vi "Sequence Anal Tri_Di.vi"(8 "Level Composition":string[](array[string]), 11 "String":string="TCTAGACTATCTCACTCTCAGATGAGATCGATAGATCAGT") -> (0 "BaseNumber":cluster{i32[], i32[], i32[]}, 1 "B%Number":cluster{dbl[], dbl[], dbl[]}, 3 "Base Tag":T1)   [LabVIEW 2018]
panel:
  out "MonoBase_Array_Tag":string[](array[string])=["AC", "AT", "AG", "CA", "CG", "CT", "GA", "GC", "GT", "TA", "TC", "TG"]
  out "MonoBase_Array":i32[](array[numeric])
  out "Mono_Array":string[](array[string])
  out "TriBase_Array":i32[](array[numeric])
  out "TriBase_Array_Tag":string[](array[string])=["AC", "AT", "AG", "CA", "CG", "CT", "GA", "GC", "GT", "TA", "TC", "TG"]
  out "DiBase_Array_Tag":string[](array[string])=["AC", "AT", "AG", "CA", "CG", "CT", "GA", "GC", "GT", "TA", "TC", "TG"]
  out "DiBase_Array":i32[](array[numeric])
  out "TriBase_Array":string[](array[string])
  out "DiBase_Array":string[](array[string])
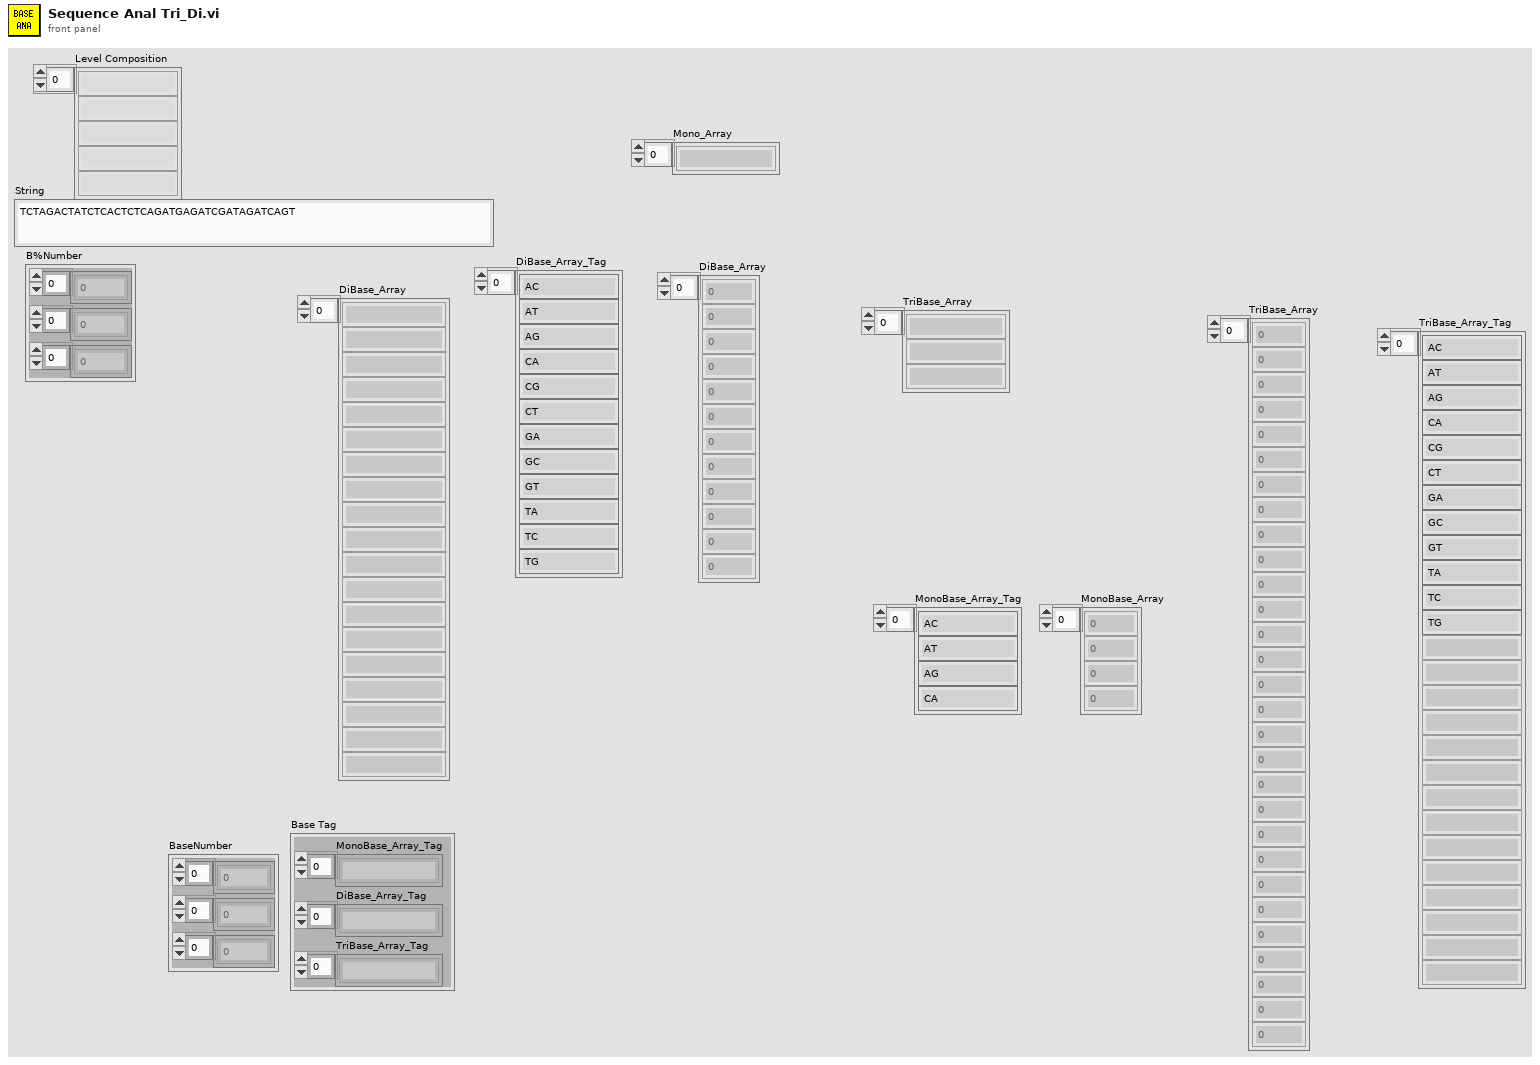
[diagram p1: front panel]
types:
  T1 = cluster{"MonoBase_Array_Tag":string[], "DiBase_Array_Tag":string[], "TriBase_Array_Tag":string[]}
  T2 = cluster{"Level Composition":string[], string[], string[]}
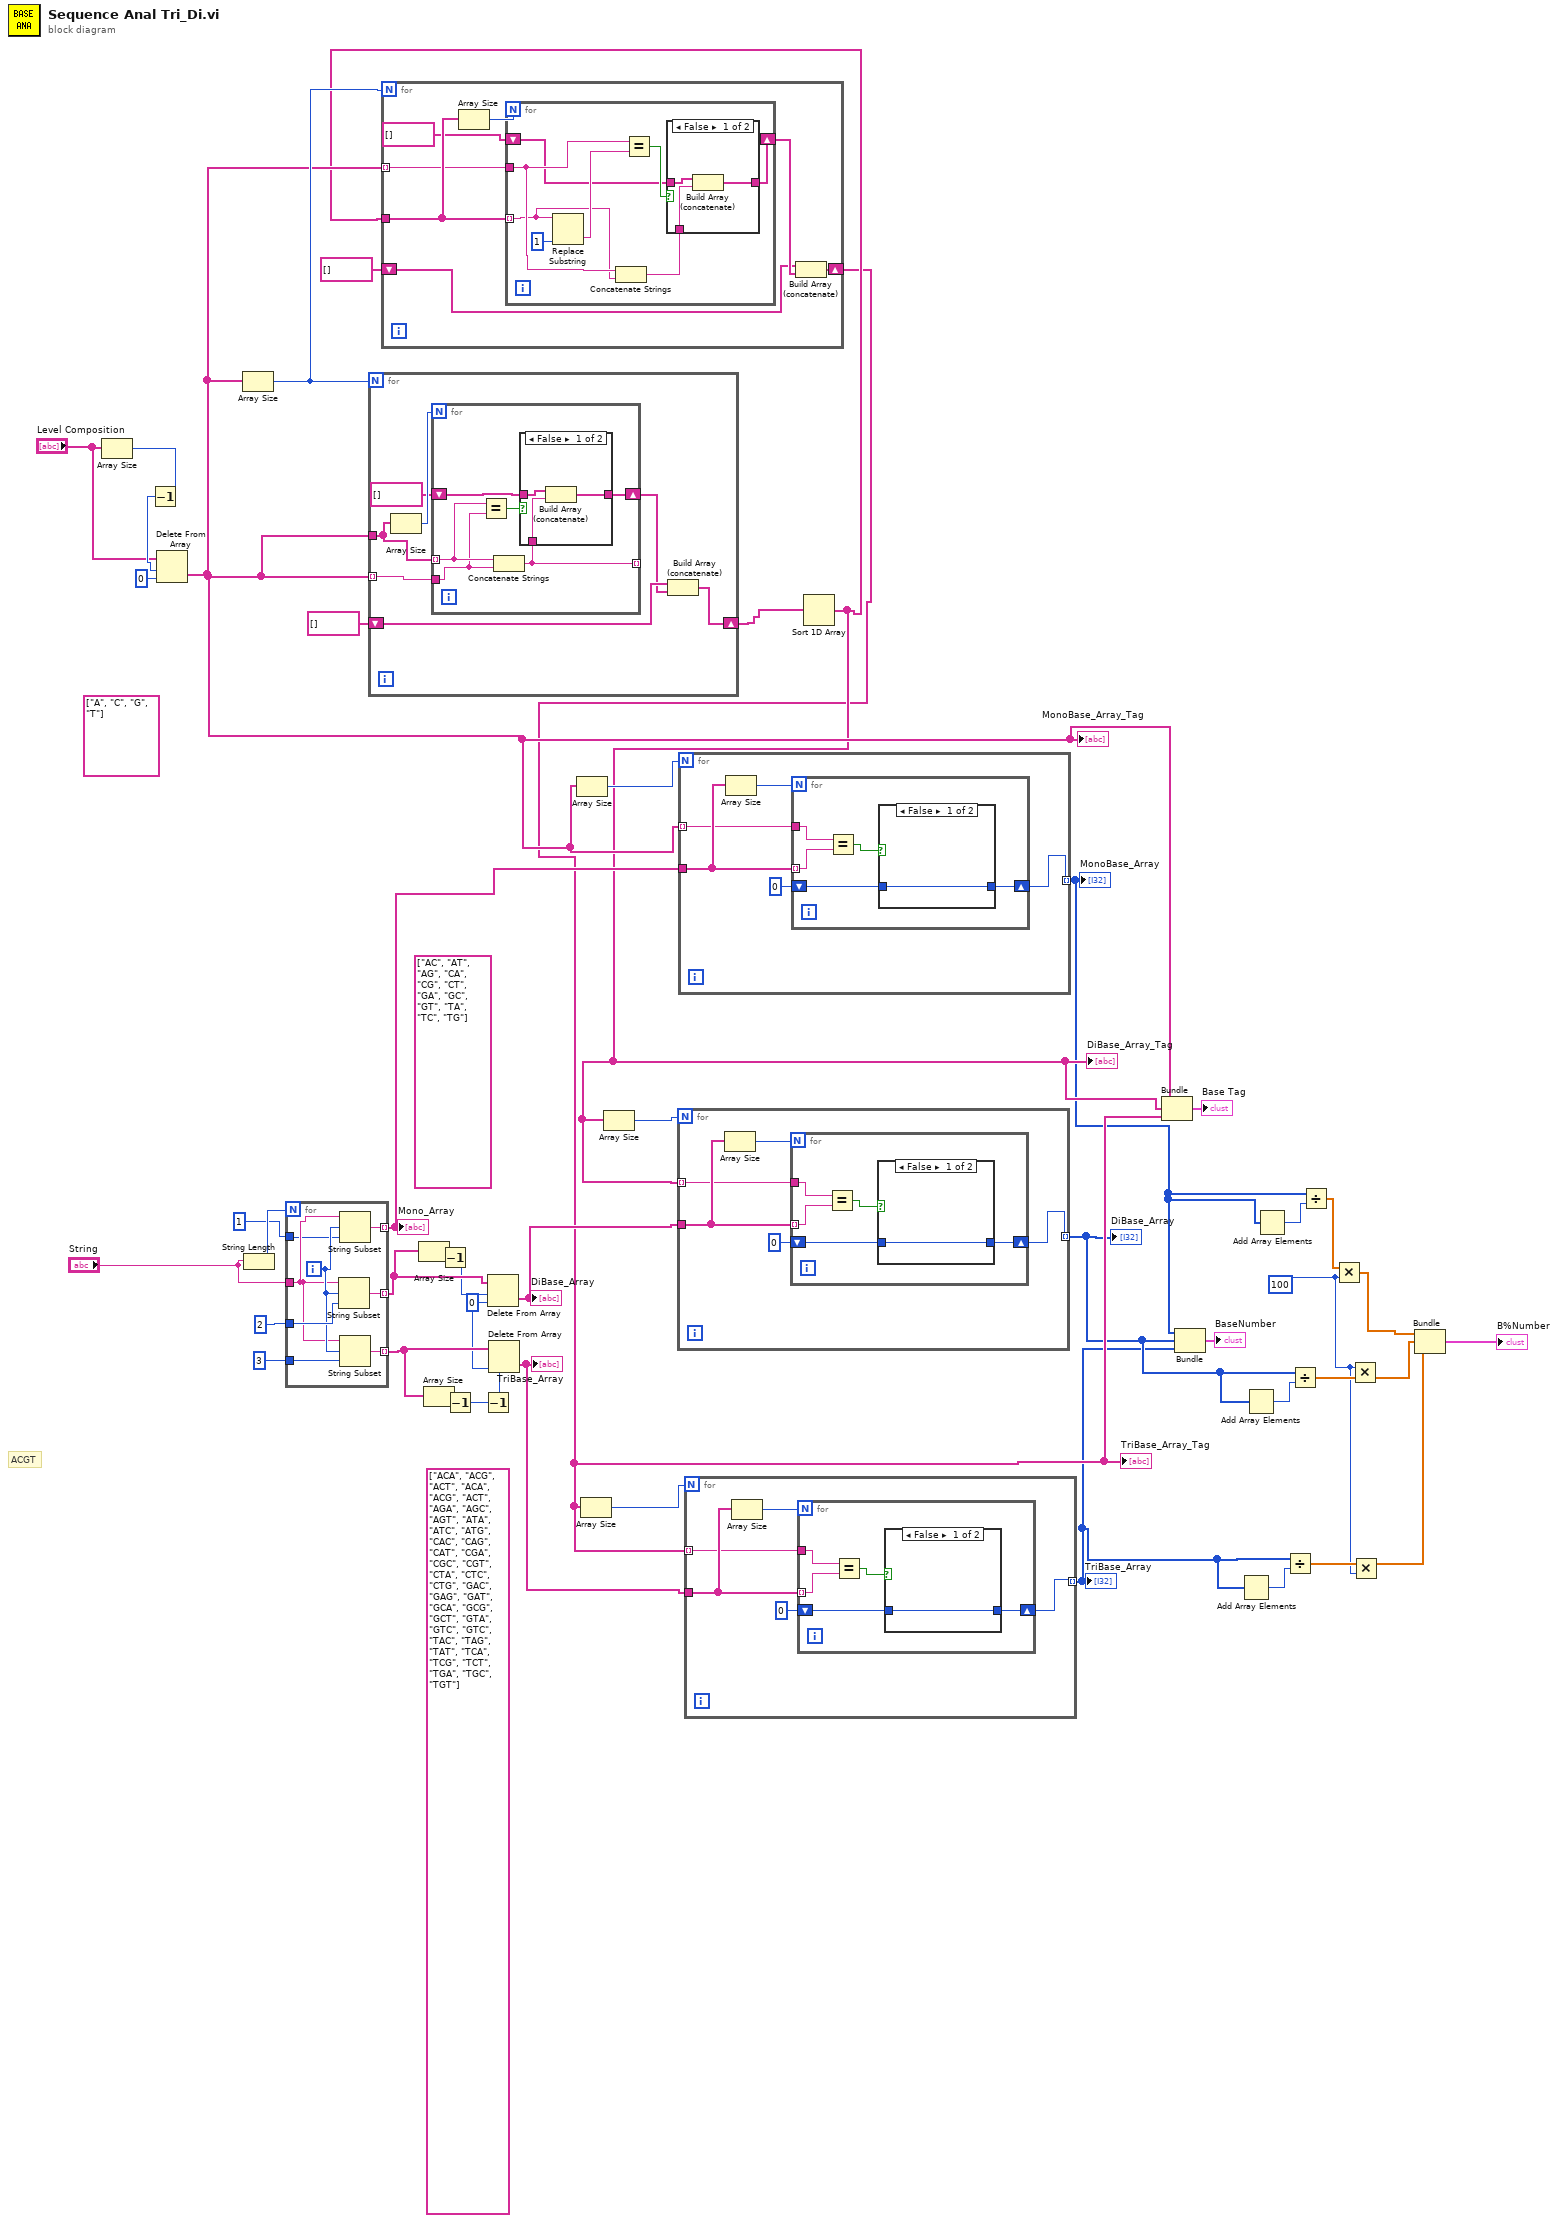
[diagram p0: block diagram]
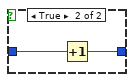
[diagram p4: hidden frame]
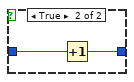
[diagram p5: hidden frame]
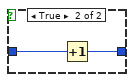
[diagram p6: hidden frame]
diagram:
  w2 = 100
  (unwired) string[] ["A", "C", "G", "T"] ("appended array")
  w36 = 0 ("index")
  (unwired) string[] ["AC", "AT", "AG", "CA", "CG", "CT", "GA", "GC", "GT", "TA", "TC", "TG"] ("appended array 2")
  (unwired) string[] ["ACA", "ACG", "ACT", "ACA", "ACG", "ACT", "AGA", "AGC", "AGT", "ATA", "ATC", "ATG", "CAC", "CAG", "CAT", "CGA", "CGC", "CGT", "CTA", "CTC", "CTG", "GAC", "GAG", "GAT", "GCA", "GCG", "GCT", "GTA", "GTC", "GTC", "TAC", "TAG", "TAT", "TCA", "TCG", "TCT", "TGA", "TGC", "TGT"] ("appended array")
  # "ACGT"
  n1 = Array Size(array="Level Composition") -> (size(s)=w23:i32)
  n2 = Decrement(x=w23) -> (x-1=w22:i32)
  n3 = Delete From Array(array="Level Composition", length=w22, index=0) -> (deleted portion=w18:string[])  [unwired: 1 out]
  "MonoBase_Array_Tag" <- w18
  n4 = Array Size(array=w18) -> (size(s)=w19:i32)
  n5 = String Length(string="String") -> (length=w46:i32)
  n6 = for {
    N: w46 -> [_]
    tunnel: "String" -> [w49]
    tunnel: [w54] -> w43 mode=indexing
    tunnel: 2 ("length (rest)") -> [w53]
    tunnel: [w52] -> w39 mode=indexing
    tunnel: 3 ("length (rest)") -> [w51]
    tunnel: 1 ("length (rest)") -> [w48]
    tunnel: [w47] -> w28 mode=indexing
    i -> [w50]
    n7 = String Subset(string=w49, offset (0)=w50, length (rest)=w53) -> (substring=w54:string)
    n8 = String Subset(string=w49, offset (0)=w50, length (rest)=w48) -> (substring=w47:string)
    n9 = String Subset(string=w49, offset (0)=w50, length (rest)=w51) -> (substring=w52:string)
  }
  "Mono_Array" <- w28
  n10 = for {
    N: w19 -> [_]
    tunnel: w18 -> [w60]
    tunnel: w18 -> [w59] mode=indexing
    shift-right: [w58] -> w20
    shift-left: string[] [] -> [w57]
    n11 = Array Size(array=w60) -> (size(s)=w61:i32)
    n12 = for {
      N: w61 -> [_]
      tunnel: w60 -> [w67] mode=indexing
      tunnel: w59 -> [w66]
      tunnel: [w64] -> _ mode=indexing
      shift-right: [w63] -> w55
      shift-left: string[] [] -> [w62]
      n13 = Equal?(x=w67, y=w66) -> (x = y?=w65:bool)
      n14 = Concatenate Strings(w67, w66) -> (w64:string)
      n15 = case shown="False" w65 {
        tunnel: w64 -> [w70 _]
        tunnel: [w69 w71] -> w63
        tunnel: w62 -> [w68 w71]
        frame False {
          n16 = Build Array (concatenate)(w68, w70) -> (w69:string[])
        }
        frame True {
        }
      }
    }
    n17 = Build Array (concatenate)(w57, w55) -> (w58:string[])
  }
  n18 = Array Size(array=w43) -> (size(s)=w42:i32)
  n19 = Array Size(array=w39) -> (size(s)=w40:i32)
  n20 = Decrement(x=w42) -> (x-1=w41:i32)
  n21 = Decrement(x=w40) -> (x-1=w38:i32)
  n22 = Decrement(x=w38) -> (x-1=w37:i32)
  n23 = Delete From Array(array=w43, length=w41, index=w36) -> (deleted portion=w33:string[])  [unwired: 1 out]
  "DiBase_Array" <- w33
  n24 = Delete From Array(array=w39, length=w37, index=w36) -> (deleted portion=w31:string[])  [unwired: 1 out]
  "TriBase_Array" <- w31
  n25 = Array Size(array=w18) -> (size(s)=w29:i32)
  n26 = for {
    N: w29 -> [_]
    tunnel: w18 -> [w74] mode=indexing
    tunnel: w28 -> [w76]
    tunnel: [w72] -> w13 mode=indexing
    n27 = Array Size(array=w76) -> (size(s)=w75:i32)
    n28 = for {
      N: w75 -> [_]
      tunnel: w76 -> [w80] mode=indexing
      tunnel: w74 -> [w81]
      shift-right: [w78] -> w72
      shift-left: 0 -> [w77]
      n29 = Equal?(x=w81, y=w80) -> (x = y?=w79:bool)
      n30 = case shown="False" w79 {
        tunnel: w77 -> [w82 w84]
        tunnel: [w82 w83] -> w78
        frame False {
        }
        frame True {
          n31 = Increment(x=w84) -> (x+1=w83:i32)
        }
      }
    }
  }
  "MonoBase_Array" <- w13
  n32 = Sort 1D Array(array=w20) -> (sorted array=w17:string[])
  "DiBase_Array_Tag" <- w17
  n33 = for {
    N: w19 -> [_]
    tunnel: w18 -> [w89] mode=indexing
    tunnel: w17 -> [w90]
    shift-right: [w86] -> w15
    shift-left: string[] [] -> [w85]
    n34 = Array Size(array=w90) -> (size(s)=w91:i32)
    n35 = for {
      N: w91 -> [_]
      tunnel: w90 -> [w93] mode=indexing
      tunnel: w89 -> [w97]
      shift-right: [w95] -> w87
      shift-left: string[] [] -> [w94]
      n36 = Replace Substring(2:1 ("length (len. of substring)"), 5:w93) -> (0:w98:string)  [unwired: 2 in, 1 out]
      n37 = Concatenate Strings(w97, w93) -> (w92:string)
      n38 = Equal?(x=w97, y=w98) -> (x = y?=w96:bool)
      n39 = case shown="False" w96 {
        tunnel: w92 -> [w102 _]
        tunnel: [w101 w103] -> w95
        tunnel: w94 -> [w100 w103]
        frame False {
          n40 = Build Array (concatenate)(w100, w102) -> (w101:string[])
        }
        frame True {
        }
      }
    }
    n41 = Build Array (concatenate)(w85, w87) -> (w86:string[])
  }
  "TriBase_Array_Tag" <- w15
  n42 = Array Size(array=w15) -> (size(s)=w32:i32)
  n43 = Array Size(array=w17) -> (size(s)=w34:i32)
  n44 = for {
    N: w34 -> [_]
    tunnel: w17 -> [w106] mode=indexing
    tunnel: w33 -> [w108]
    tunnel: [w104] -> w9 mode=indexing
    n45 = Array Size(array=w108) -> (size(s)=w107:i32)
    n46 = for {
      N: w107 -> [_]
      tunnel: w108 -> [w112] mode=indexing
      tunnel: w106 -> [w113]
      shift-right: [w110] -> w104
      shift-left: 0 -> [w109]
      n47 = Equal?(x=w113, y=w112) -> (x = y?=w111:bool)
      n48 = case shown="False" w111 {
        tunnel: w109 -> [w114 w116]
        tunnel: [w114 w115] -> w110
        frame False {
        }
        frame True {
          n49 = Increment(x=w116) -> (x+1=w115:i32)
        }
      }
    }
  }
  "DiBase_Array" <- w9
  n50 = for {
    N: w32 -> [_]
    tunnel: w15 -> [w119] mode=indexing
    tunnel: w31 -> [w121]
    tunnel: [w117] -> w7 mode=indexing
    n51 = Array Size(array=w121) -> (size(s)=w120:i32)
    n52 = for {
      N: w120 -> [_]
      tunnel: w121 -> [w125] mode=indexing
      tunnel: w119 -> [w126]
      shift-right: [w123] -> w117
      shift-left: 0 -> [w122]
      n53 = Equal?(x=w126, y=w125) -> (x = y?=w124:bool)
      n54 = case shown="False" w124 {
        tunnel: w122 -> [w127 w129]
        tunnel: [w127 w128] -> w123
        frame False {
        }
        frame True {
          n55 = Increment(x=w129) -> (x+1=w128:i32)
        }
      }
    }
  }
  "TriBase_Array" <- w7
  n56 = Bundle("Level Composition"=w18, w17, w15) -> (→"Base Tag":T2)  [unwired: 1 in]
  n57 = Bundle(w13, w9, w7) -> (→"BaseNumber":cluster{i32[], i32[], i32[]})  [unwired: 1 in]
  n58 = Add Array Elements(numeric array=w7) -> (sum=w8:i32)
  n59 = Add Array Elements(numeric array=w9) -> (sum=w11:i32)
  n60 = Add Array Elements(numeric array=w13) -> (sum=w14:i32)
  n61 = Divide(x=w7, y=w8) -> (x/y=w4:dbl[])
  n62 = Divide(x=w9, y=w11) -> (x/y=w10:dbl[])
  n63 = Divide(x=w13, y=w14) -> (x/y=w12:dbl[])
  n64 = Multiply(x=w12, y=w2) -> (x*y=w6:dbl[])
  n65 = Multiply(x=w2, y=w10) -> (x*y=w5:dbl[])
  n66 = Multiply(x=w4, y=w2) -> (x*y=w3:dbl[])
  n67 = Bundle(w6, w5, w3) -> (→"B%Number":cluster{dbl[], dbl[], dbl[]})  [unwired: 1 in]
